vi "Temp_Sensor_test.vi"() -> ()   [LabVIEW 2026]
panel:
  in  "stop":bool
  out "Boolean":bool
  out "Waveform Chart":dbl(graph)
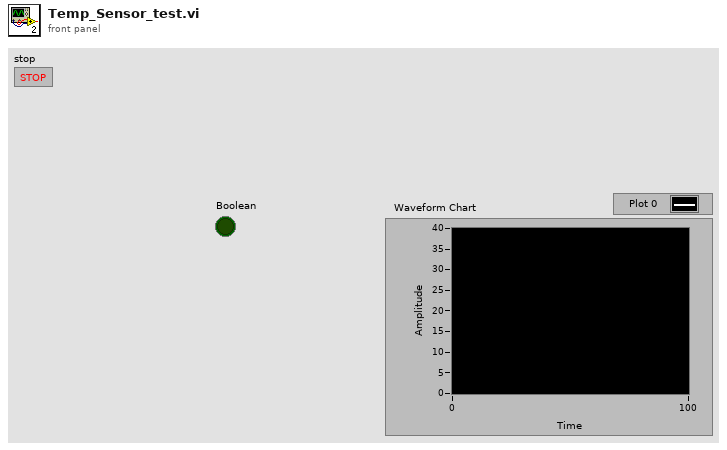
[diagram p1: front panel]
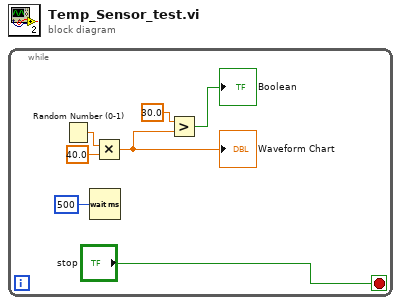
[diagram p0: block diagram]
diagram:
  n1 = while {
    stop <- "stop" stop-if-true
    n2 = Random Number (0-1)() -> (number: 0 to 1=w5:dbl)
    n3 = Wait (ms)(milliseconds to wait=u32 500) -> ()  [unwired: 1 out]
    n4 = Multiply(x=w5, y=40.0) -> (x*y=w4:dbl)
    "Waveform Chart" <- w4
    n5 = Greater?(x=30.0, y=w4) -> (0:→"Boolean":bool)
  }
